vi "Find_GT_File_Path.vi"(8 "error in":errorcluster, 10 "GT Mask Folder Path":path=path "D:/DNN/MVTec/pill/ground_truth", 11 "Image File Path":path=path "D:/DNN/MVTec/pill/ground_truth") -> (0 "error out":errorcluster, 1 "Found?":bool, 2 "GT File Path":path, 3 "Image File Path out":path=path "D:/DNN/MVTec/pill/ground_truth")   [LabVIEW 2020]
panel:
  out "Progress":i32
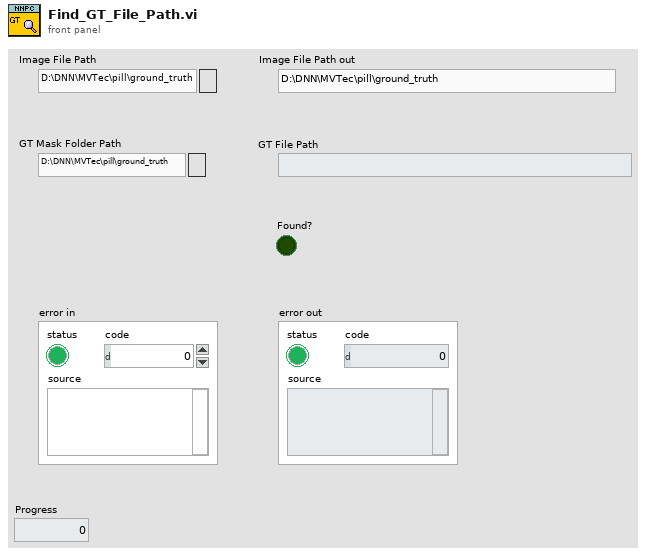
[diagram p1: front panel]
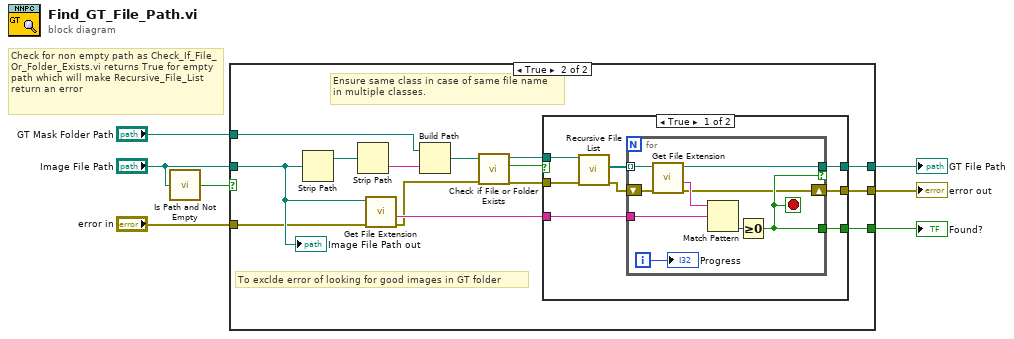
[diagram p0: block diagram]
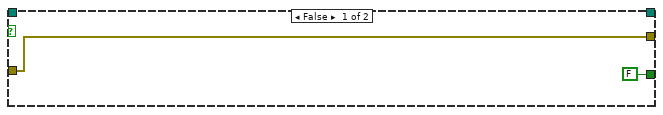
[diagram p2: hidden frame]
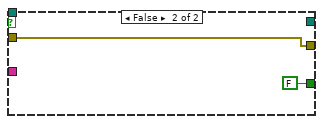
[diagram p3: hidden frame]
diagram:
  # "Check for non empty path as Check_If_File_Or_Folder_Exists.vi returns True for empty path which will make Recursive_File_List return an error"
  n1 = call <vilib>:"Is Path and Not Empty.vi"("path"="Image File Path") -> ("Is Path and Not Empty?"=w1:bool)  [unwired: 4 in]
  n2 = case shown="True" w1 {
    tunnel: "Image File Path" -> [_ w21]
    tunnel: [_ w19] -> w7
    tunnel: [FALSE w18] -> w6
    tunnel: [w9 w17] -> w5
    tunnel: "error in" -> [w9 w16]
    tunnel: "GT Mask Folder Path" -> [_ w10]
    frame False {
    }
    frame True {
      # "To exclde error of looking for good images in GT folder"
      # "Ensure same class in case of same file name\nin multiple classes."
      n3 = Strip Path(path=w21) -> (stripped path=w23:path)  [unwired: 1 out]
      n4 = Strip Path(path=w23) -> (name=w22:string)  [unwired: 1 out]
      n5 = call <vilib>:"Get File Extension.vi"("error in (no error)"=w16, "file"=w21) -> ("error out"=w15:errorcluster, "filename without extension"=w20:string)  [unwired: 5 in, 3 out]
      n6 = Build Path(base path=w10, name or relative path=w22) -> (appended path=w14:path)
      n7 = call <vilib>:"Check if File or Folder Exists.vi"("error in (no error)"=w15, "path"=w14) -> ("error out"=w12:errorcluster, "file or folder exists?"=w11:bool, "dup path"=w13:path)  [unwired: 7 in]
      n8 = case shown="True" w11 {
        tunnel: w20 -> [w31 _]
        tunnel: [w30 _] -> w19
        tunnel: [w29 FALSE] -> w18
        tunnel: [w26 w42] -> w17
        tunnel: w13 -> [w25 _]
        tunnel: w12 -> [w24 w42]
        frame True {
          n9 = call <vilib>:"Recursive File List.vi"("error in (no error)"=w24, "Folder Path"=w25) -> ("error out"=w27:errorcluster, "All Files in Dir"=w28:path[])  [unwired: 5 in, 3 out]
          n10 = for {
            tunnel: w28 -> [w37] mode=indexing
            tunnel: w31 -> [w40]
            tunnel: [w36] -> w30 if=w35
            tunnel: [w35] -> w29
            shift-right: [w33] -> w26
            shift-left: w27 -> [w34]
            i -> [w32]
            stop <- w35 stop-if-true
            n11 = call <vilib>:"Get File Extension.vi"("error in (no error)"=w34, "file"=w37) -> ("error out"=w33:errorcluster, "filename without extension"=w38:string, "dup file"=w36:path)  [unwired: 5 in, 2 out]
            n12 = Match Pattern(string=w38, regular expression=w40) -> (offset past match=w39:i32)  [unwired: 1 in, 3 out]
            n13 = Greater Or Equal To 0?(x=w39) -> (x >= 0?=w35:bool)
            "Progress" <- w32
          }
        }
        frame False {
        }
      }
      "Image File Path out" <- w21
    }
  }
  "GT File Path" <- w7
  "Found?" <- w6
  "error out" <- w5
